vi "strings to memory.vi"(8 "error in":errorcluster, 11 "1.0.0":T1) -> (0 "error out":errorcluster, 3 "memory hierarchy":T5)   [LabVIEW 2014, in "NISE_CEF_TreeSerializer.lvlib"]
doc: "Unflattens a flattened instance data hierarchy into an object hierarchy."
uses:
  NISE_CEF_TreeSerializer.lvlib
  memory hierarchy.ctl
  full hierarchy.ctl
  hierarchy element.ctl
  serializable configuration/NISE_CEF_serializable configuration.lvclass
  flat hierarchy.ctl
  instance data.ctl
  class discovery singleton/class discovery singleton methods.ctl
  class discovery singleton/class discovery singleton.lvlib
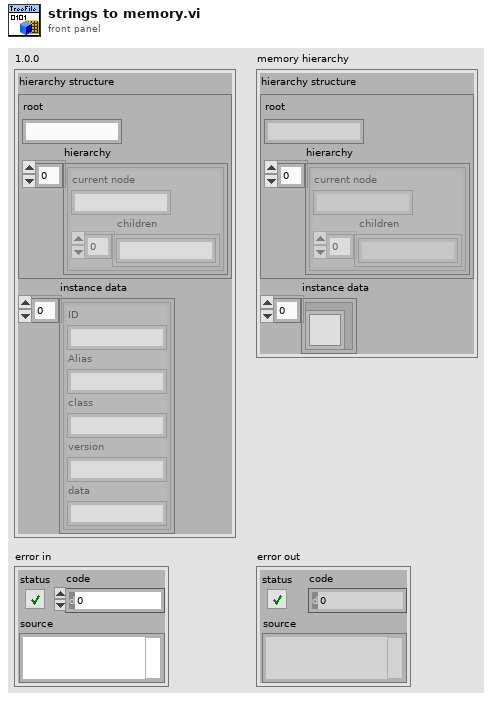
[diagram p1: front panel]
types:
  T1 = typedef "NISE_CEF_TreeSerializer.lvlib/flat hierarchy.ctl" = cluster{"hierarchy structure":T2, "instance data":T4[]}
  T2 = typedef "NISE_CEF_TreeSerializer.lvlib/full hierarchy.ctl" = cluster{"root":string, "hierarchy":T3[]}
  T3 = typedef "NISE_CEF_TreeSerializer.lvlib/hierarchy element.ctl" = cluster{"current node":string, "children":string[]}
  T4 = typedef "NISE_CEF_TreeSerializer.lvlib/instance data.ctl" = cluster{"ID":string, "Alias":string, "class":string, "version":string, "data":string}
  T5 = typedef "NISE_CEF_TreeSerializer.lvlib/memory hierarchy.ctl" = cluster{"hierarchy structure":T2, "instance data":refnum<class "NISE_CEF_serializable configuration.lvclass">[]}
  T6 = typedef "class discovery singleton.lvlib/class discovery singleton methods.ctl" = enum16{"add search paths", "load class by name", "list available classes", "get class path", "delete cache"}
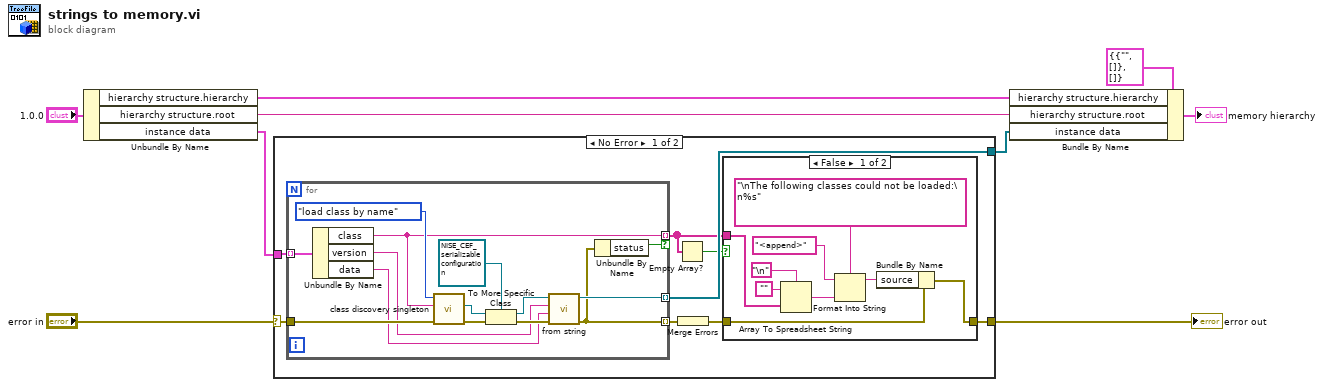
[diagram p0: block diagram]
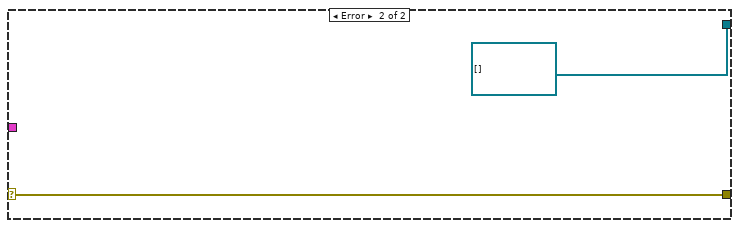
[diagram p3: hidden frame]
diagram:
  n1 = Unbundle By Name("1.0.0") -> ("hierarchy structure.hierarchy"=w4:T3[], "hierarchy structure.root"=w5:string, "instance data"=w3:T4[])
  n2 = case shown="No Error" "error in" {
    selector: "error in" -> [w10 w43]
    tunnel: [w17 w43] -> w7
    tunnel: w3 -> [w16 _]
    tunnel: [w15 refnum<class "NISE_CEF_serializable configuration.lvclass">[] []] -> w2
    frame No Error {
      n3 = for {
        tunnel: w16 -> [w31] mode=indexing
        tunnel: [w23] -> w15 mode=indexing
        tunnel: w10 -> [w26]
        tunnel: [w19] -> w11 mode=indexing
        tunnel: [w20] -> w12 mode=indexing if=w18
        n4 = Unbundle By Name(w31) -> ("class"=w20:string, "version"=w21:string, "data"=w22:string)
        n5 = call "class discovery singleton.vi"("error in"=w26, "Class Name"=w20, "method"=class_discovery_singleton_methods."load class by name") -> ("error out"=w29:errorcluster, "LabVIEW Object"=w28:refnum<class>)  [unwired: 5 in, 2 out]
        n6 = To More Specific Class(target class=refnum<class "NISE_CEF_serializable configuration.lvclass"> refnum ("configuration in"), reference=w28, error in=w29) -> (specific class reference=w24:refnum<class "NISE_CEF_serializable configuration.lvclass">, error out=w25:errorcluster)
        n7 = call-dynamic "from string.vi"("error in"=w25, "data"=w22, "version"=w21, "configuration in"=w24) -> ("error out"=w19:errorcluster, "configuration out"=w23:refnum<class "NISE_CEF_serializable configuration.lvclass">)  [unwired: 6 in]
        n8 = Unbundle By Name(w19) -> ("status"=w18:bool)
      }
      n9 = Empty Array?(array=w12) -> (empty?=w14:bool)
      n10 = Merge Errors(w11) -> (w13:errorcluster)
      n11 = case shown="False" w14 {
        tunnel: w13 -> [w40 w41]
        tunnel: [w39 w41] -> w17
        tunnel: w12 -> [w33 _]
        frame False {
          n12 = Array To Spreadsheet String(delimiter (Tab)="\n", array=w33, 3:"" ("format string")) -> (spreadsheet string=w35:string)
          n13 = Format Into String(format string="\nThe following classes could not be loaded:\n%s", initial string="<append>", w35) -> (resulting string=w34:string)  [unwired: 1 in, 1 out]
          n14 = Bundle By Name(cluster=w40, "source"=w34) -> (w39:errorcluster)
        }
        frame True {
        }
      }
    }
    frame Error {
    }
  }
  "error out" <- w7
  n15 = Bundle By Name(cluster=T5 {"hierarchy structure"={"root"="", "hierarchy"=[]}, "instance data"=[]} ("memory hierarchy"), "hierarchy structure.hierarchy"=w4, "hierarchy structure.root"=w5, "instance data"=w2) -> (→"memory hierarchy":T5)
